vi "CSL UI.vi"() -> ()   [LabVIEW 2025, in "CSL.lvlib" / "CSL.lvclass"]
doc: "Copyright 2017 National Instruments Corporation\n\nLicensed under the Apache License, Version 2.0 (the \"License\"); you may not use this file except in compliance with the License. You may obtain a copy of the License at http://www.apache.org/licenses/LICENSE-2.0\nUnless required by applicable law or agreed to in writing, software distributed under the License is distributed on an \"AS IS\" BASIS, WITHOUT WARRANTIES OR CONDITIONS OF ANY KIND, either express or implied. See the License for the specific language governing permissions and limitations under the License."
uses:
  CSL.lvclass
  CSL.lvclass/CSL.ctl
  C:/Users/Public/Documents/Sandia National Labs/TSS Plugin/CEF.lvlibp/serializable node/CEF_serializable node.lvclass
  C:/Users/Public/Documents/Sandia National Labs/TSS Plugin/CEF.lvlibp/Node/CEF_Node.lvclass
  C:/Working copy/TS Manager/Plugin/Core Setting Layer/CSL/CSL/CSL.lvclass
  Users/Public/Documents/Sandia National Labs/TSS Plugin/CEF.lvlibp/Node/CEF_Node.lvclass
  CSL configuration/CSL configuration.lvclass
  Users/Public/Documents/Sandia National Labs/TSS Plugin/CEF.lvlibp/Node/UserEventRef.ctl
  Users/Public/Documents/Sandia National Labs/TSS Plugin/CEF.lvlibp/Node/mainQref.ctl
  Users/Public/Documents/Sandia National Labs/TSS Plugin/CEF.lvlibp/Node/NodeRef.ctl
  CSL configuration/Test Info.ctl
panel:
  in  "node ref":T1
  in  "CSL":T2={"General"={"Operator"="JLee"}}
  in  "main queue":T3
  in  "user event":T4
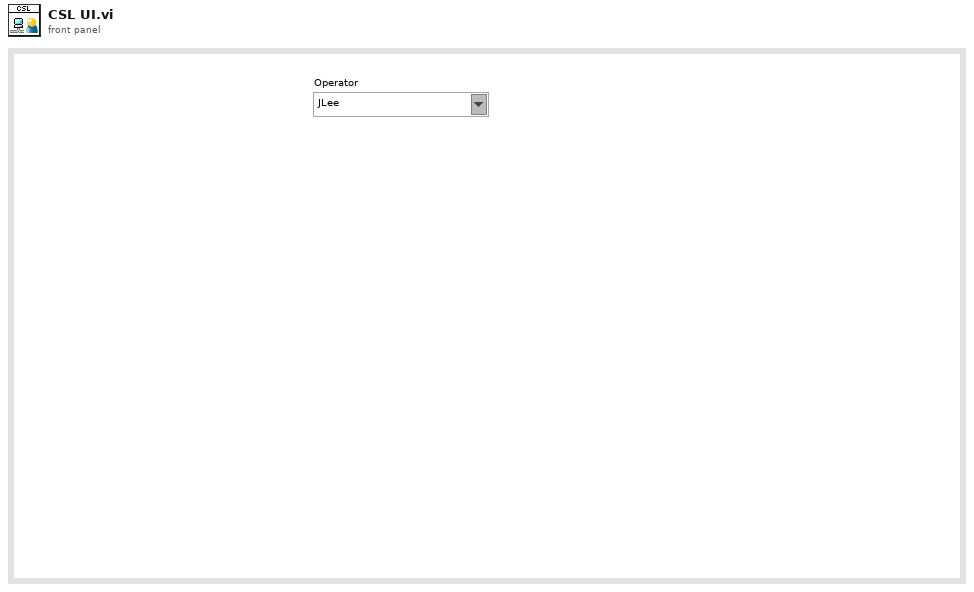
[diagram p1: front panel]
types:
  T1 = typedef "CEF.lvlibp/CEF_Node.lvclass/NodeRef.ctl" = refnum<data-value>
  T2 = typedef "CSL.lvlib/CSL configuration.lvclass/Test Info.ctl" = cluster{"General":cluster{"Operator":string}}
  T3 = typedef "CEF.lvlibp/CEF_Node.lvclass/mainQref.ctl" = refnum<queue>
  T4 = typedef "CEF.lvlibp/CEF_Node.lvclass/UserEventRef.ctl" = refnum<user-event>
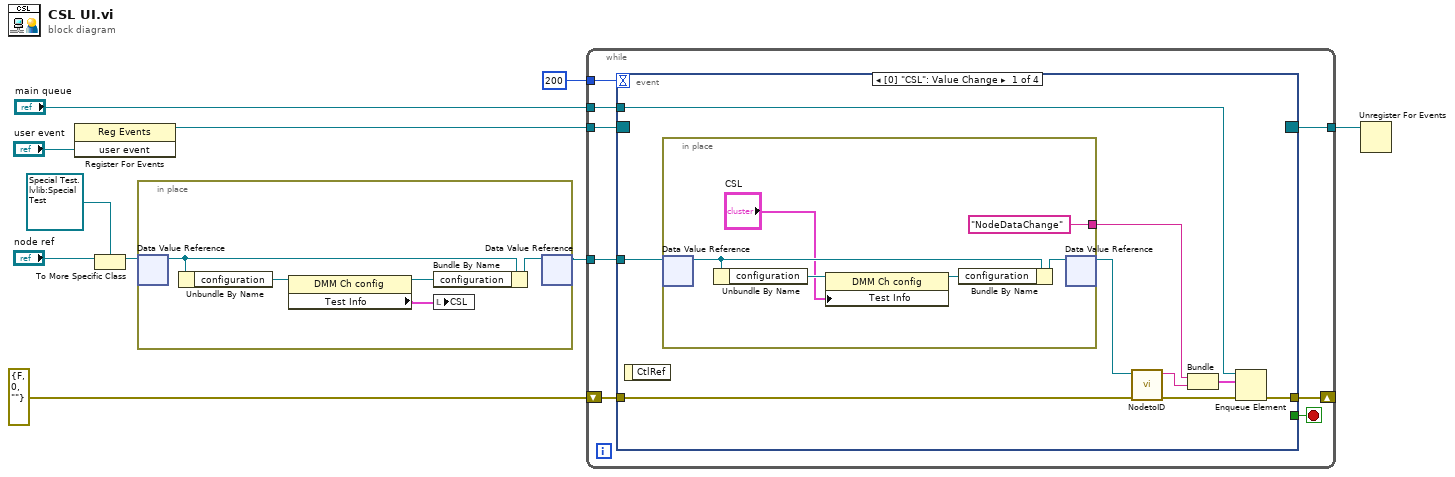
[diagram p0: block diagram]
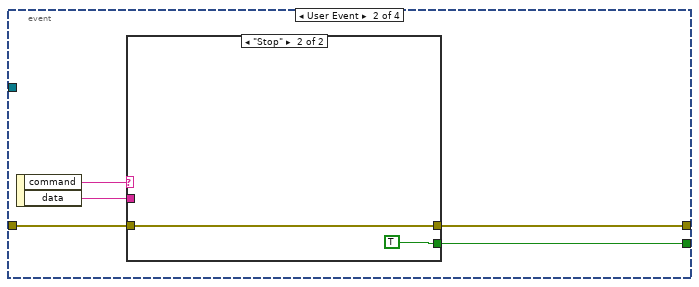
[diagram p2: hidden frame]
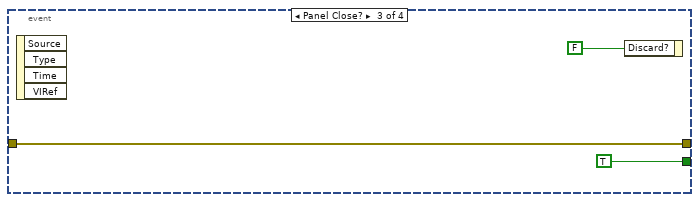
[diagram p4: hidden frame]
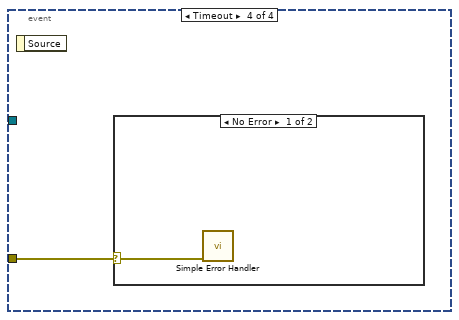
[diagram p5: hidden frame]
diagram:
  n1 = register-events("user event") -> (reference out=w9:refnum<event-registration>)  [unwired: 2 in, 1 out]
  n2 = To More Specific Class(target class=refnum<data-value> refnum ("data value reference"), reference="node ref") -> (specific class reference=w5:refnum<data-value>)  [unwired: 1 in, 1 out]
  n3 = in-place {
    # "Initialize the front panel controls when loaded"
    n4 = in-place-dvr #1(w5) -> (w15:refnum<class "CSL.lvclass">)  [unwired: 1 out]
    n5 = Unbundle By Name(w15) -> ("configuration"=w14:refnum<class "CSL configuration.lvclass">)
    n6 = property class="DMM Ch config"(reference=w14) -> (reference out=w12:refnum<class "CSL configuration.lvclass">, "Test Info"=w11:T2)  [unwired: 1 in, 1 out]
    n7 = Bundle By Name(cluster=w15, "configuration"=w12) -> (w13:refnum<class "CSL.lvclass">)
    n8 = local write "CSL"(w11) -> ()
    n9 = in-place-dvr #1(w13) -> (w4:refnum<data-value>)  [unwired: 1 out]
  }
  n10 = while {
    tunnel: w9 -> [w23]
    tunnel: [w22] -> w8
    shift-right: [w20] -> _
    shift-left: errorcluster {"status"=FALSE, "code"=0, "source"=""} ("error in (no error)") -> [w19]
    tunnel: "main queue" -> [w18]
    tunnel: w4 -> [w17]
    tunnel: 200 -> [w16]
    stop <- w21 stop-if-true
    n11 = event shown="[0] \"CSL\": Value Change" {
      selector: w23 -> [_ _ _ _]
      dyn-events: [_ _ _ _] -> w22
      timeout: w16 -> [_ _ _ _]
      tunnel: [_ w43 TRUE _] -> w21
      tunnel: [w27 w41 w48 _] -> w20
      tunnel: w19 -> [w28 w42 w48 w50]
      tunnel: w18 -> [w26 _ _ _]
      tunnel: w17 -> [w32 _ _ _]
      event Value Change {
        n12 = event-data() -> ()  [unwired: 1 in, 1 out]
        n13 = in-place {
          in-place-border: ["NodeDataChange" ("Message Name")] -> w25
          n14 = in-place-dvr #2(w32) -> (w38:refnum<class "CSL.lvclass">)  [unwired: 1 out]
          n15 = Unbundle By Name(w38) -> ("configuration"=w35:refnum<class "CSL configuration.lvclass">)
          n16 = property class="DMM Ch config"(reference=w35, "Test Info"="CSL") -> (reference out=w37:refnum<class "CSL configuration.lvclass">)  [unwired: 1 in, 1 out]
          n17 = Bundle By Name(cluster=w38, "configuration"=w37) -> (w36:refnum<class "CSL.lvclass">)
          n18 = in-place-dvr #2(w36) -> (w24:refnum<data-value>)  [unwired: 1 out]
        }
        n19 = call "NodetoID.vi"("error in"=w28, "node ref"=w24) -> ("error out"=w31:errorcluster, "ID"=w29:string)  [unwired: 8 in]
        n20 = Bundle("Message Name"=w25, "ID"=w29) -> (w30:cluster{"Message Name":string, "ID":string})  [unwired: 1 in]
        n21 = Enqueue Element(queue=w26, element=w30, error in (no error)=w31) -> (error out=w27:errorcluster)  [unwired: 1 in, 2 out]
      }
      event User Event {
        n22 = event-data() -> ("command"=w39:string, "data"=w40:string)  [unwired: 1 in]
        n23 = case shown="\"Stop\"" w39 {
          tunnel: w40 -> [_ _]
          tunnel: [_ TRUE] -> w43
          tunnel: w42 -> [w44 w45]
          tunnel: [w44 w45] -> w41
          frame Default {
          }
          frame "Stop" {
          }
        }
      }
      event Panel Close? {
        n24 = event-data() -> ()  [unwired: 1 in, 4 out]
        n25 = event-data("Discard?"=FALSE) -> ()  [unwired: 1 in, 1 out]
      }
      event Timeout {
        n26 = event-data() -> ()  [unwired: 1 in, 1 out]
        n27 = case shown="No Error" w50 {
          selector: w50 -> [w51 _]
          frame No Error {
            n28 = call <vilib>:"Simple Error Handler.vi"("error in (no error)"=w51) -> ()  [unwired: 4 in, 5 out]
          }
          frame Error {
          }
        }
      }
    }
  }
  n29 = Unregister For Events(event registration refnum=w8) -> ()  [unwired: 1 in, 1 out]
